vi "Indexer.vi"() -> ()   [LabVIEW 2020]
doc: "Use this template to build a producer/consumer design pattern with events to produce queue items. Use this design pattern instead of the User Interface Event Handler pattern for user interfaces when you want to execute code asynchronously in response to an event without slowing the user interface responsiveness."
uses:
  Model/AbstractModel/AbstractModel.lvclass
  Model/MarkovModel/MarkovModel.lvclass
  C:/Projects/DMC/DMC-Complete/Model/AbstractModel/AbstractModel.lvclass
  DBMap/DBMap.lvclass
  DBSet/DBSet.lvclass
  Indexer Action.ctl
  File Metadata.ctl
  Node.ctl
  Source to Sink Array.ctl
  File Data.ctl
panel:
  out "data":T5
  in  "Tab Control":enum32{"Main", "Debug"}(tab)
  in  "Download Pre-Index Button":bool
  out "# of files":i32 format="%d files"
  out "Markov Progress":u64(slide) scale=-1.0..4743.0
  out "Saving model to file":bool
  in  "Run Training":bool
  in  "Training Folders":path[](array[path])
  in  "Load Example Paths":bool
  out "Pulling training files":bool
  out "Converting to node-child maps":bool
  out "Training model":bool
  out "Node Progress":u64(slide) scale=-1.0..10515.0
  in  "stop":bool
  in  "Load from file":bool
  in  "Save to file":bool
  in  "Stage 3 - Train Model":bool
  in  "Stage 1 - Pull Example Files":bool
  in  "Stage 2 - Convert to Node-Child Maps":bool
  in  "Parallel Instances":i32=8
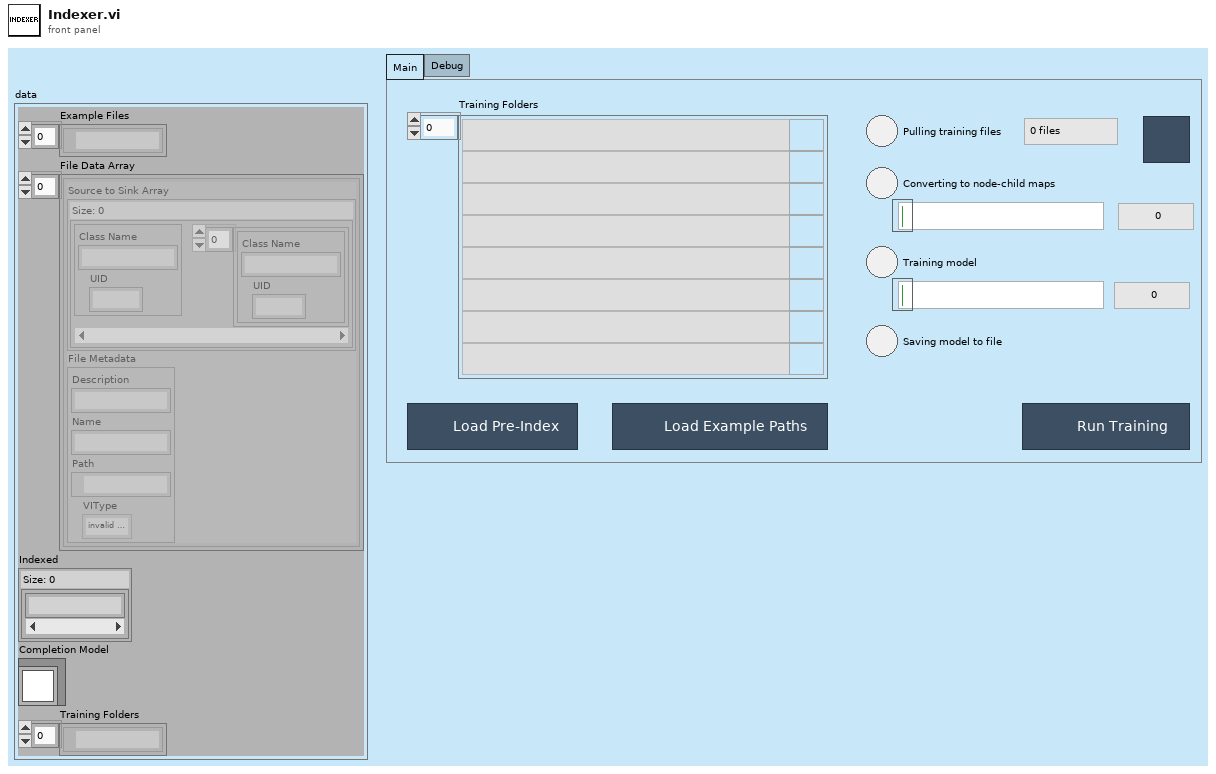
[diagram p1: front panel]
types:
  T1 = typedef "File Data.ctl" = cluster{"Source to Sink Array":T2, "File Metadata":T4}
  T2 = typedef "Source to Sink Array.ctl" = map{T3, T3[]}
  T3 = typedef "Node.ctl" = cluster{"Class Name":string, "UID":i32}
  T4 = typedef "File Metadata.ctl" = cluster{"Description":string, "Name":string, "Path":path, "VIType":enum32{"invalid VI type", "Standard VI", "Control VI", "Global VI", "Polymorphic VI", "Configuration VI", "SubSystem", "Facade VI", "Method VI", "Statechart Diagram VI"}}
  T5 = cluster{"Example Files":path[], "File Data Array":T1[], "Indexed":set{string}, "Completion Model":refnum<class "AbstractModel.lvclass">, "Training Folders":path[]}
  T6 = typedef "Indexer Action.ctl" = enum16{"Pull Training Files", "Convert to Node-Child Maps", "Train Model", "Save to file", "Load from file", "Load Example Paths", "Download Pre-Index"}
  T7 = enum8{"Enabled", "Disabled", "Disabled and Grayed Out"}
  T8 = cluster{"Example Files":path[], "File Data Array":T1[], "Indexed":set{string}, "MarkovModel out":refnum<class "MarkovModel.lvclass">, "Training Folders":path[]}
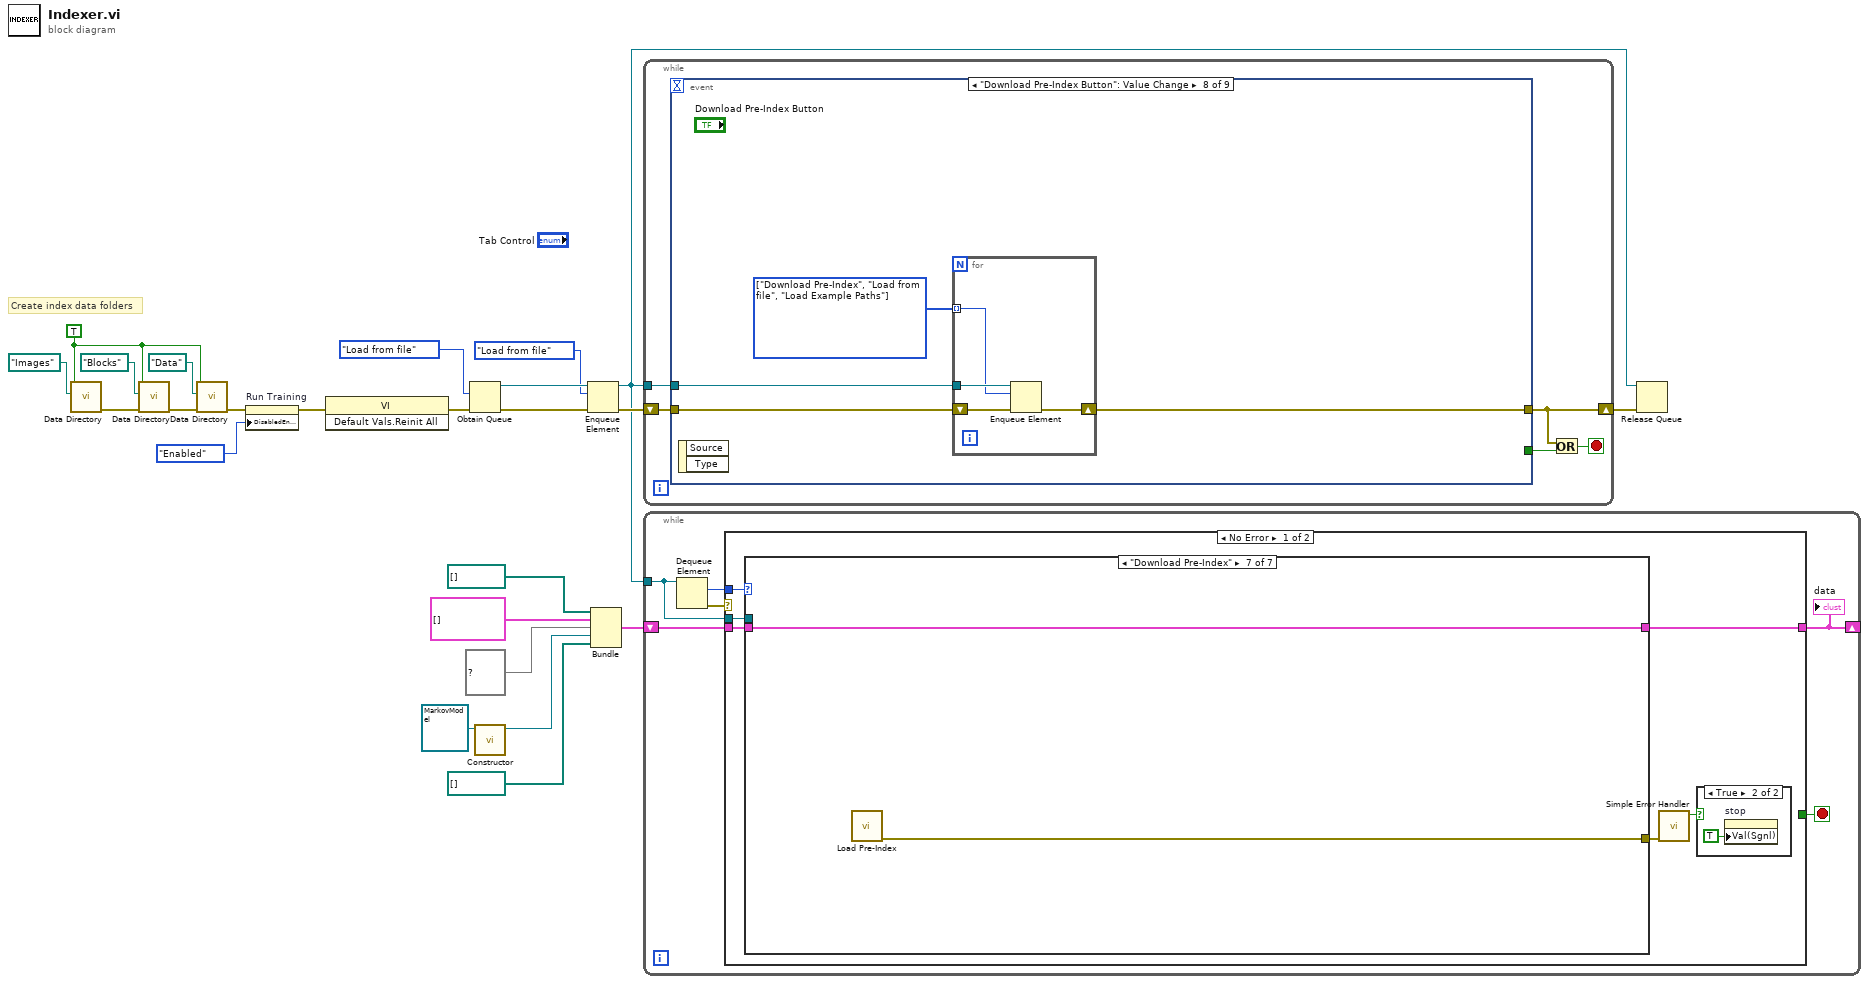
[diagram p0: block diagram]
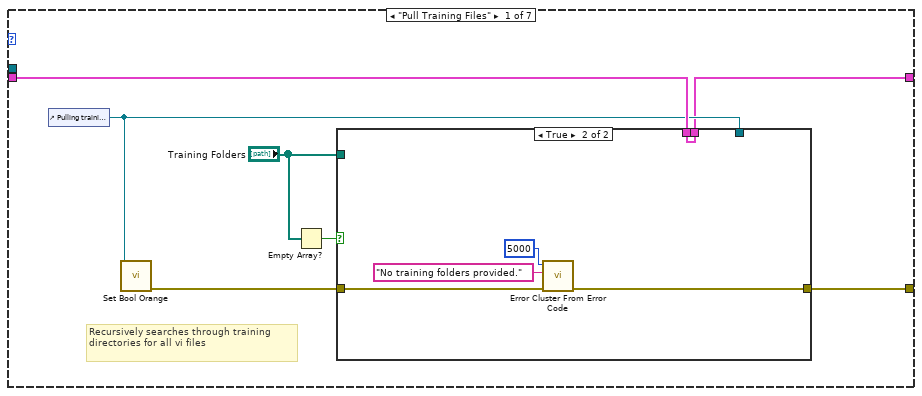
[diagram p2: hidden frame]
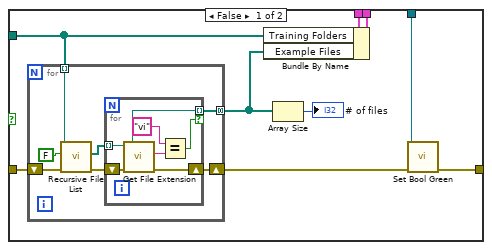
[diagram p3: hidden frame]
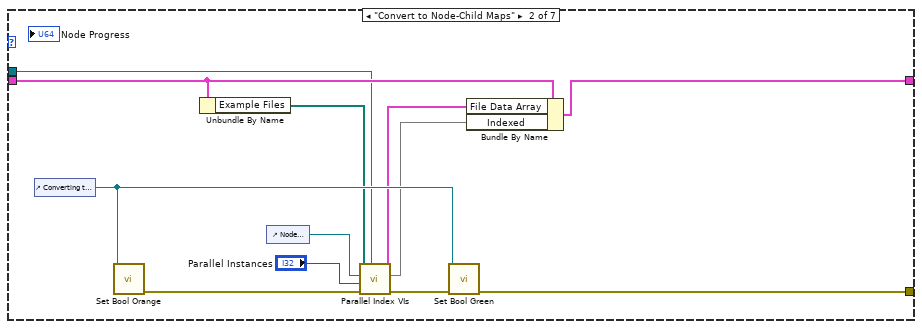
[diagram p4: hidden frame]
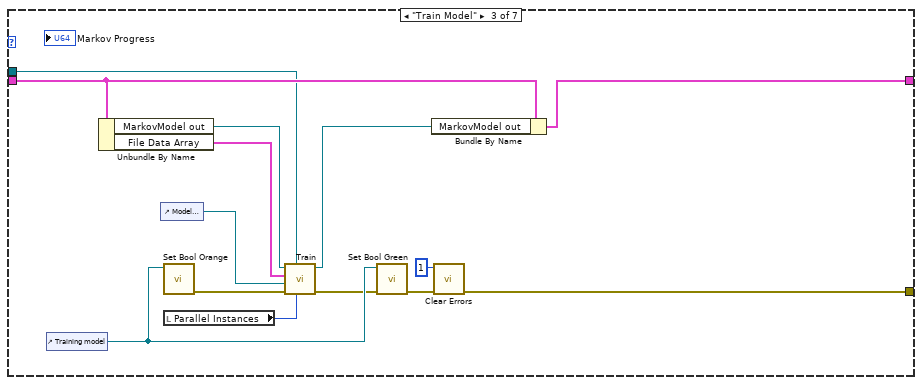
[diagram p5: hidden frame]
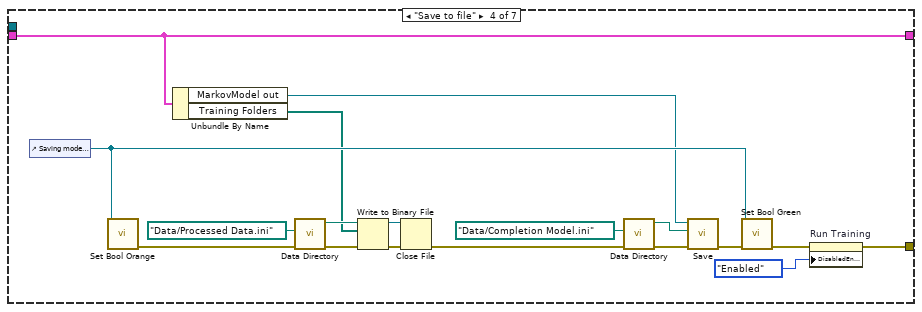
[diagram p6: hidden frame]
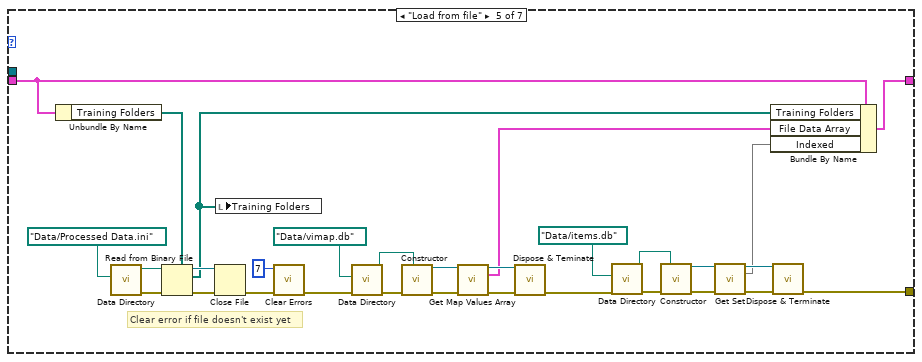
[diagram p7: hidden frame]
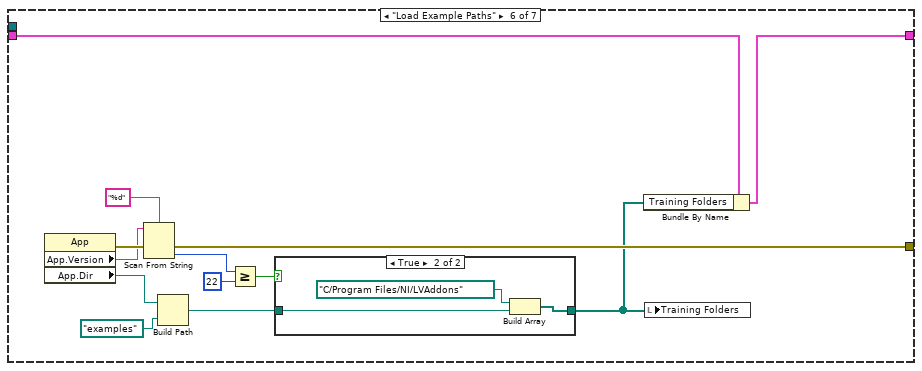
[diagram p8: hidden frame]
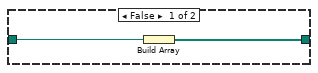
[diagram p9: hidden frame]
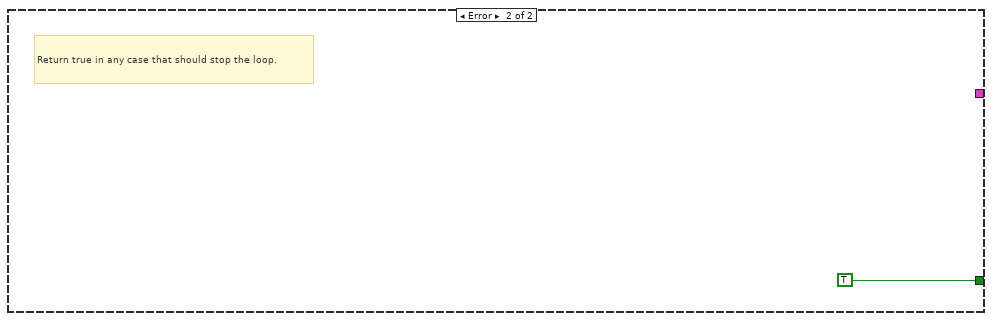
[diagram p11: hidden frame]
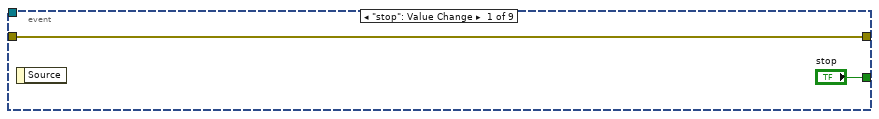
[diagram p12: hidden frame]
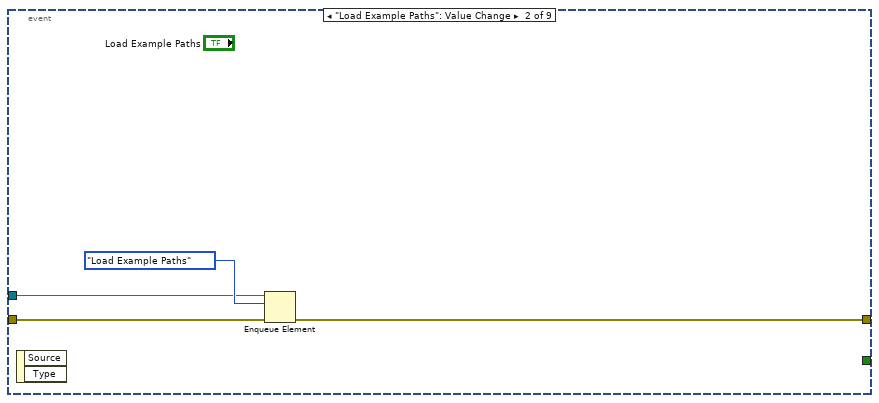
[diagram p13: hidden frame]
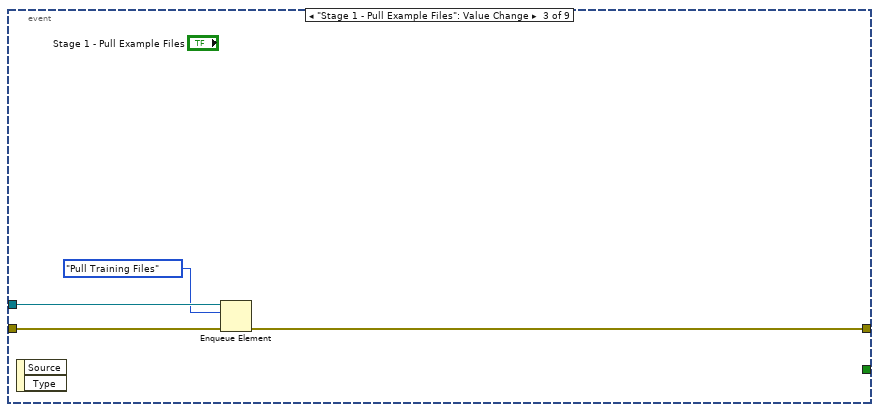
[diagram p14: hidden frame]
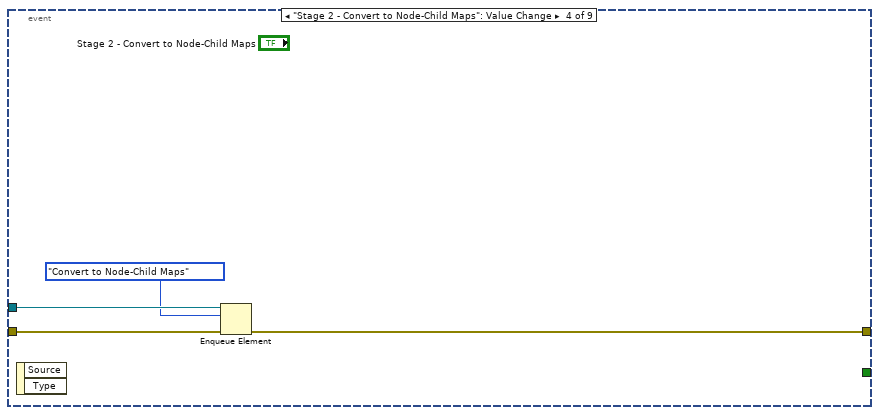
[diagram p15: hidden frame]
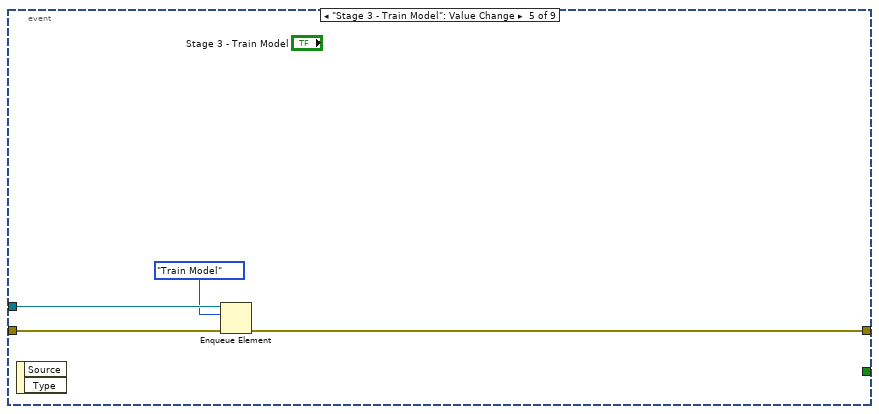
[diagram p16: hidden frame]
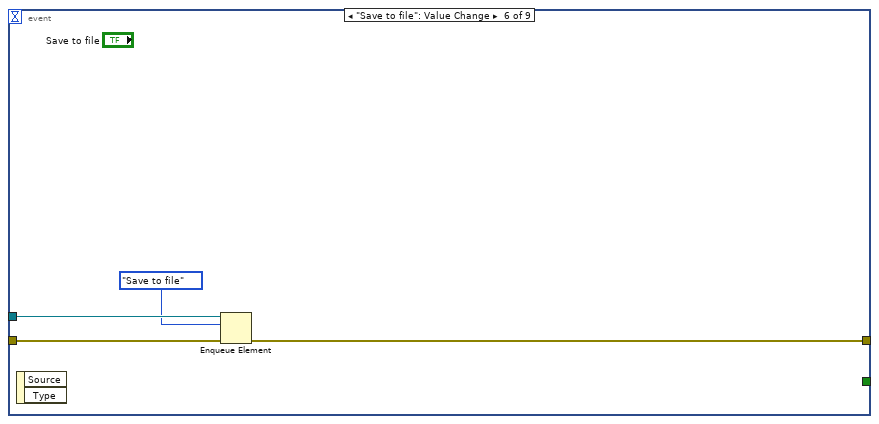
[diagram p17: hidden frame]
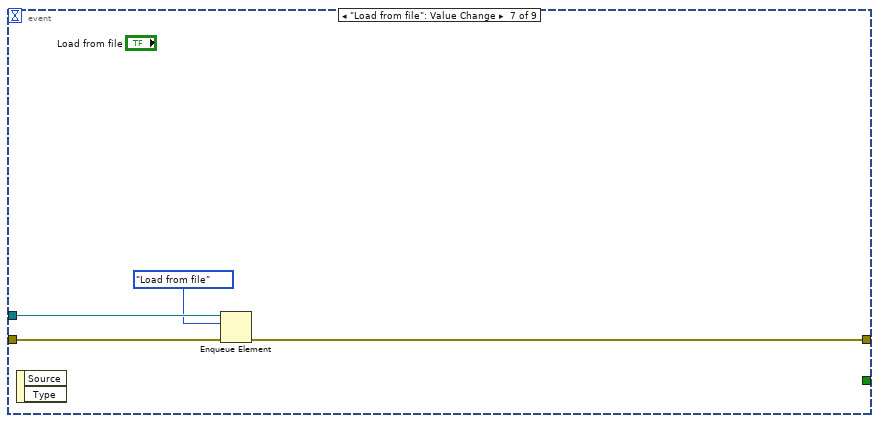
[diagram p18: hidden frame]
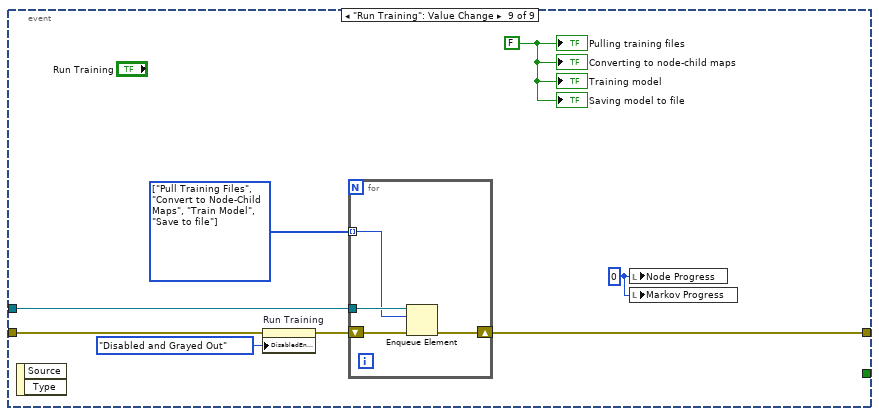
[diagram p19: hidden frame]
diagram:
  w5 = TRUE ("Create if doesn't exist? (F)")
  # "Create index data folders"
  n1 = call "Data Directory.vi"("Subdirectory"=path "Images" ("name or relative path"), "Create if doesn't exist? (F)"=w5) -> ("error out"=w6:errorcluster)  [unwired: 8 in, 1 out]
  n2 = call "Data Directory.vi"("error in (no error)"=w6, "Subdirectory"=path "Blocks" ("name or relative path"), "Create if doesn't exist? (F)"=w5) -> ("error out"=w7:errorcluster)  [unwired: 7 in, 1 out]
  n3 = call "Data Directory.vi"("error in (no error)"=w7, "Subdirectory"=path "Data" ("name or relative path"), "Create if doesn't exist? (F)"=w5) -> ("error out"=w4:errorcluster)  [unwired: 7 in, 1 out]
  n4 = property on="Run Training" class="Bool"(error in=w4, "DisabledEnum"=T7."Enabled") -> (error out=w12:errorcluster)  [unwired: 1 in, 1 out]
  n5 = invoke class="VI" method="Default Vals.Reinit All"(error in=w12) -> (error out=w14:errorcluster)  [unwired: 2 in, 2 out]
  n6 = Obtain Queue(element data type=Indexer_Action."Load from file" ("Indexer Action"), error in (no error)=w14) -> (queue out=w17:refnum<queue>, error out=w19:errorcluster)  [unwired: 3 in, 1 out]
  n7 = call-dynamic "Constructor.vi"("MarkovModel in"=refnum<class "MarkovModel.lvclass"> refnum ("MarkovModel.lvclass")) -> ("MarkovModel out"=w1:refnum<class "MarkovModel.lvclass">)  [unwired: 9 in, 1 out]
  n8 = Enqueue Element(queue=w17, element=Indexer_Action."Load from file", error in (no error)=w19) -> (queue out=w15:refnum<queue>, error out=w18:errorcluster)  [unwired: 1 in, 1 out]
  n9 = Bundle("Example Files"=path[] [], "File Data Array"=T1[] [], "Indexed"=set{string} {}, "MarkovModel out"=w1, "Training Folders"=path[] []) -> (w20:T8)  [unwired: 1 in]
  n10 = while {
    shift-right: [w25] -> w24
    shift-left: w18 -> [w28]
    tunnel: w15 -> [w29]
    stop <- w26 stop-if-true
    n11 = event shown="[7] \"Download Pre-Index Button\": Value Change" {
      selector: _ -> [_ _ _ _ _ _ _ _ _]
      dyn-events: _ -> [_ _ _ _ _ _ _ _ _]
      timeout: _ -> [_ _ _ _ _ _ _ _ _]
      tunnel: w29 -> [_ w32 w38 w42 w46 w50 w54 w57 w71]
      tunnel: w28 -> [w30 w34 w39 w43 w47 w51 w55 w59 w67]
      tunnel: [w30 w33 w37 w41 w45 w49 w53 w58 w70] -> w25
      tunnel: ["stop" _ _ _ _ _ _ _ _] -> w27
      event "stop": Value Change {
        n12 = event-data() -> ()  [unwired: 1 in, 1 out]
      }
      event "Load Example Paths": Value Change {
        n13 = event-data() -> ()  [unwired: 1 in, 2 out]
        n14 = Enqueue Element(queue=w32, element=Indexer_Action."Load Example Paths" ("Indexer Action"), error in (no error)=w34) -> (error out=w33:errorcluster)  [unwired: 1 in, 2 out]
      }
      event "Stage 1 - Pull Example Files": Value Change {
        n15 = event-data() -> ()  [unwired: 1 in, 2 out]
        n16 = Enqueue Element(queue=w38, element=Indexer_Action."Pull Training Files" ("Indexer Action"), error in (no error)=w39) -> (error out=w37:errorcluster)  [unwired: 1 in, 2 out]
      }
      event "Stage 2 - Convert to Node-Child Maps": Value Change {
        n17 = event-data() -> ()  [unwired: 1 in, 2 out]
        n18 = Enqueue Element(queue=w42, element=Indexer_Action."Convert to Node-Child Maps" ("Indexer Action"), error in (no error)=w43) -> (error out=w41:errorcluster)  [unwired: 1 in, 2 out]
      }
      event "Stage 3 - Train Model": Value Change {
        n19 = event-data() -> ()  [unwired: 1 in, 2 out]
        n20 = Enqueue Element(queue=w46, element=Indexer_Action."Train Model" ("Indexer Action"), error in (no error)=w47) -> (error out=w45:errorcluster)  [unwired: 1 in, 2 out]
      }
      event "Save to file": Value Change {
        n21 = event-data() -> ()  [unwired: 1 in, 2 out]
        n22 = Enqueue Element(queue=w50, element=Indexer_Action."Save to file" ("Indexer Action"), error in (no error)=w51) -> (error out=w49:errorcluster)  [unwired: 1 in, 2 out]
      }
      event "Load from file": Value Change {
        n23 = event-data() -> ()  [unwired: 1 in, 2 out]
        n24 = Enqueue Element(queue=w54, element=Indexer_Action."Load from file" ("Indexer Action"), error in (no error)=w55) -> (error out=w53:errorcluster)  [unwired: 1 in, 2 out]
      }
      event "Download Pre-Index Button": Value Change {
        w56 = T6[] [enum."Download Pre-Index", enum."Load from file", enum."Load Example Paths"] items=["Pull Training Files", "Convert to Node-Child Maps", "Train Model", "Save to file", "Load from file", "Load Example Paths", "Download Pre-Index"] ("Array")
        n25 = event-data() -> ()  [unwired: 1 in, 2 out]
        n26 = for {
          tunnel: w57 -> [w62]
          tunnel: w56 -> [w60] mode=indexing
          shift-right: [w61] -> w58
          shift-left: w59 -> [w63]
          n27 = Enqueue Element(queue=w62, element=w60, error in (no error)=w63) -> (error out=w61:errorcluster)  [unwired: 1 in, 2 out]
        }
      }
      event "Run Training": Value Change {
        w64 = u64 0 ("Node Progress")
        w65 = FALSE ("Pulling training files")
        w69 = T6[] [enum."Pull Training Files", enum."Convert to Node-Child Maps", enum."Train Model", enum."Save to file"] items=["Pull Training Files", "Convert to Node-Child Maps", "Train Model", "Save to file", "Load from file", "Load Example Paths", "Download Pre-Index"] ("Array")
        n28 = event-data() -> ()  [unwired: 1 in, 2 out]
        n29 = property on="Run Training" class="Bool"(error in=w67, "DisabledEnum"=T7."Disabled and Grayed Out" ("Disabled")) -> (error out=w68:errorcluster)  [unwired: 1 in, 1 out]
        n30 = for {
          tunnel: w71 -> [w74]
          tunnel: w69 -> [w72] mode=indexing
          shift-right: [w73] -> w70
          shift-left: w68 -> [w75]
          n31 = Enqueue Element(queue=w74, element=w72, error in (no error)=w75) -> (error out=w73:errorcluster)  [unwired: 1 in, 2 out]
        }
        n32 = local write "Node Progress"(w64) -> ()
        n33 = local write "Markov Progress"(w64) -> ()
        "Converting to node-child maps" <- w65
        "Training model" <- w65
        "Pulling training files" <- w65
        "Saving model to file" <- w65
      }
    }
    n34 = Or(x=w25, y=w27) -> (x .or. y?=w26:bool)
  }
  n35 = while {
    tunnel: w15 -> [w77]
    shift-right: [w76] -> _
    shift-left: w20 -> [w78]
    stop <- w79 stop-if-true
    n36 = Dequeue Element(queue=w77) -> (element=w80:T6, error out=w81:errorcluster)  [unwired: 2 in, 2 out]
    n37 = case shown="No Error" w81 {
      tunnel: w80 -> [w87 _]
      tunnel: [_ TRUE] -> w79
      tunnel: w78 -> [w86 _]
      tunnel: [w85 _] -> w76
      tunnel: w77 -> [w84 _]
      frame No Error {
        n38 = case shown="\"Download Pre-Index\"" w87 {
          tunnel: [w88 w122 w134 w151 w186 w197 w214] -> w85
          tunnel: w86 -> [w94 w133 w146 w151 w188 w198 w214]
          tunnel: w84 -> [_ w127 w140 _ _ _ _]
          tunnel: [w92 w131 w144 w160 w166 w200 w215] -> w83
          frame "Pull Training Files" {
            # "Recursively searches through training directories for all vi files"
            n39 = control-ref of="Pulling training files"() -> (w91:refnum<vi>)
            n40 = call "Set Bool Orange.vi"("Indicator ref in"=w91) -> ("error out"=w93:errorcluster)  [unwired: 10 in]
            n41 = Empty Array?(array="Training Folders") -> (empty?=w89:bool)
            n42 = case shown="True" w89 {
              tunnel: w94 -> [w103 w121]
              tunnel: [w102 w121] -> w88
              tunnel: w93 -> [w101 w120]
              tunnel: [w99 w119] -> w92
              tunnel: w91 -> [w98 _]
              tunnel: "Training Folders" -> [w95 _]
              frame False {
                n43 = for {
                  tunnel: w95 -> [w110] mode=indexing
                  shift-right: [w105] -> w100
                  shift-left: w101 -> [w106]
                  tunnel: [w104] -> w97 mode=concatenating
                  n44 = call <vilib>:"Recursive File List.vi"("error in (no error)"=w106, "Treat LLBs as Folders?"=FALSE, "Folder Path"=w110) -> ("error out"=w107:errorcluster, "All Files in Dir"=w108:path[])  [unwired: 4 in, 3 out]
                  n45 = for {
                    tunnel: w108 -> [w113] mode=indexing
                    tunnel: [w113] -> w104 mode=indexing if=w112
                    shift-right: [w111] -> w105
                    shift-left: w107 -> [w116]
                    n46 = call <vilib>:"Get File Extension.vi"("error in (no error)"=w116, "file"=w113) -> ("error out"=w111:errorcluster, "lowercase file extension"=w114:string)  [unwired: 5 in, 3 out]
                    n47 = Equal?(x="vi", y=w114) -> (x = y?=w112:bool)
                  }
                }
                n48 = Bundle By Name(cluster=w103, "Training Folders"=w95, "Example Files"=w97) -> (w102:T8)
                n49 = Array Size(array=w97) -> (size(s)=→"# of files":i32)
                n50 = call "Set Bool Green.vi"("error in (no error)"=w100, "Indicator ref in"=w98) -> ("error out"=w99:errorcluster)  [unwired: 9 in]
              }
              frame True {
                n51 = call <vilib>:"Error Cluster From Error Code.vi"("error in (no error)"=w120, "error message (\"\")"="No training folders provided." ("error message (\"\")"), "error code (0)"=5000) -> ("error out"=w119:errorcluster)  [unwired: 6 in]
              }
            }
          }
          frame "Convert to Node-Child Maps" {
            n52 = control-ref of="Converting to node-child maps"() -> (w130:refnum<vi>)
            n53 = call "Set Bool Orange.vi"("Indicator ref in"=w130) -> ("error out"=w132:errorcluster)  [unwired: 10 in]
            n54 = Unbundle By Name(w133) -> ("Example Files"=w128:path[])
            n55 = control-ref of="Node Progress"() -> (w126:refnum<vi>)
            n56 = call "Parallel Index VIs.vi"("Queue in"=w127, "error in (no error)"=w132, "Parallel Instances (8)"="Parallel Instances", "Node Progress ref"=w126, "Example Files"=w128) -> ("error out"=w129:errorcluster, "Indexed"=w125:set{string}, "File Data Array"=w123:T1[])  [unwired: 4 in]
            n57 = call "Set Bool Green.vi"("error in (no error)"=w129, "Indicator ref in"=w130) -> ("error out"=w131:errorcluster)  [unwired: 9 in]
            n58 = Bundle By Name(cluster=w133, "File Data Array"=w123, "Indexed"=w125) -> (w122:T8)
          }
          frame "Train Model" {
            n59 = control-ref of="Training model"() -> (w147:refnum<vi>)
            n60 = Unbundle By Name(w146) -> ("MarkovModel out"=w139:refnum<class "MarkovModel.lvclass">, "File Data Array"=w138:T1[])
            n61 = control-ref of="Model Progress"() -> (w137:refnum<vi>)
            n62 = call "Set Bool Orange.vi"("Indicator ref in"=w147) -> ("error out"=w142:errorcluster)  [unwired: 10 in]
            n63 = local read "Parallel Instances"() -> (w136:i32)
            n64 = call-dynamic "Train.vi"("Parallel Instances (8)"=w136, "Queue in"=w140, "error in (no error)"=w142, "Progress ref in"=w137, "File Data Array"=w138, "MarkovModel in"=w139) -> ("error out"=w141:errorcluster, "MarkovModel out"=w135:refnum<class "MarkovModel.lvclass">)  [unwired: 4 in]
            n65 = call "Set Bool Green.vi"("error in (no error)"=w141, "Indicator ref in"=w147) -> ("error out"=w145:errorcluster)  [unwired: 9 in]
            n66 = Bundle By Name(cluster=w146, "MarkovModel out"=w135) -> (w134:T8)
            n67 = call <vilib>:"Clear Errors.vi"("error in (no error)"=w145, "specific error code to clear (0: all)"=1) -> ("error out"=w144:errorcluster)  [unwired: 4 in, 1 out]
          }
          frame "Save to file" {
            n68 = control-ref of="Saving model to file"() -> (w163:refnum<vi>)
            n69 = call "Set Bool Orange.vi"("Indicator ref in"=w163) -> ("error out"=w149:errorcluster)  [unwired: 10 in]
            n70 = Unbundle By Name(w151) -> ("MarkovModel out"=w156:refnum<class "MarkovModel.lvclass">, "Training Folders"=w150:path[])
            n71 = call "Data Directory.vi"("error in (no error)"=w149, "Subdirectory"=path "Data/Processed Data.ini" ("name or relative path")) -> ("error out"=w148:errorcluster, "Data directory"=w158:path)  [unwired: 8 in]
            n72 = Write to Binary File(file (use dialog)=w158, data=w150, error in=w148) -> (refnum out=w164:refnum<file>, error out=w165:errorcluster)  [unwired: 3 in, 1 out]
            n73 = Close File(refnum=w164, error in=w165) -> (error out=w153:errorcluster)  [unwired: 1 out]
            n74 = call "Data Directory.vi"("error in (no error)"=w153, "Subdirectory"=path "Data/Completion Model.ini" ("name or relative path")) -> ("error out"=w152:errorcluster, "Data directory"=w154:path)  [unwired: 8 in]
            n75 = call-dynamic "Save.vi"("error in (no error)"=w152, "Model Path"=w154, "MarkovModel in"=w156) -> ("error out"=w157:errorcluster)  [unwired: 7 in, 1 out]
            n76 = call "Set Bool Green.vi"("error in (no error)"=w157, "Indicator ref in"=w163) -> ("error out"=w161:errorcluster)  [unwired: 9 in]
            n77 = property on="Run Training" class="Bool"(error in=w161, "DisabledEnum"=T7."Enabled" ("Disabled")) -> (error out=w160:errorcluster)  [unwired: 1 in, 1 out]
          }
          frame "Load from file" {
            # "Clear error if file doesn't exist yet"
            n78 = Unbundle By Name(w188) -> ("Training Folders"=w187:path[])
            n79 = call "Data Directory.vi"("Subdirectory"=path "Data/Processed Data.ini" ("name or relative path")) -> ("error out"=w189:errorcluster, "Data directory"=w190:path)  [unwired: 9 in]
            n80 = Read from Binary File(5:w187, 8:w189, 11:w190) -> (0:w195:errorcluster, 2:w185:path[], 3:w194:refnum<file>)  [unwired: 3 in, 1 out]
            n81 = Close File(refnum=w194, error in=w195) -> (error out=w193:errorcluster)  [unwired: 1 out]
            n82 = local write "Training Folders"(w185) -> ()
            n83 = call <vilib>:"Clear Errors.vi"("error in (no error)"=w193, "specific error code to clear (0: all)"=7) -> ("error out"=w178:errorcluster)  [unwired: 4 in, 1 out]
            n84 = call "Data Directory.vi"("error in (no error)"=w178, "Subdirectory"=path "Data/vimap.db" ("name or relative path")) -> ("error out"=w183:errorcluster, "Data directory"=w182:path)  [unwired: 8 in]
            n85 = call "Constructor.vi"("SQLite DB Path"=w182, "error in (no error)"=w183) -> ("error out"=w176:errorcluster, "DBMap out"=w177:refnum<class "DBMap.lvclass">)  [unwired: 8 in]
            n86 = call "Get Map Values Array.vi"("DBMap in"=w177, "error in (no error)"=w176) -> ("DBMap out"=w174:refnum<class "DBMap.lvclass">, "File Data Array"=w172:T1[], "error out"=w175:errorcluster)  [unwired: 11 in]
            n87 = call-dynamic "Dispose & Teminate.vi"("DBMap in"=w174, "error in (no error)"=w175) -> ("error out"=w173:errorcluster)  [unwired: 12 in, 1 out]
            n88 = call "Data Directory.vi"("error in (no error)"=w173, "Subdirectory"=path "Data/items.db" ("name or relative path")) -> ("error out"=w180:errorcluster, "Data directory"=w179:path)  [unwired: 8 in]
            n89 = call "Constructor.vi"("SQLite DB Path"=w179, "error in (no error)"=w180) -> ("DBSet out"=w168:refnum<class "DBSet.lvclass">, "error out"=w171:errorcluster)  [unwired: 12 in]
            n90 = call "Get Set.vi"("DBSet in"=w168, "error in (no error)"=w171) -> ("DBSet out"=w169:refnum<class "DBSet.lvclass">, "Set"=w167:set{string}, "error out"=w170:errorcluster)  [unwired: 11 in]
            n91 = Bundle By Name(cluster=w188, "Training Folders"=w185, "File Data Array"=w172, "Indexed"=w167) -> (w186:T8)
            n92 = call-dynamic "Dispose & Terminate.vi"("DBSet in"=w169, "error in (no error)"=w170) -> ("error out"=w166:errorcluster)  [unwired: 12 in, 1 out]
          }
          frame "Load Example Paths" {
            n93 = property class="App"() -> (error out=w203:errorcluster, "App.Version"=w199:string, "App.Dir"=w204:path)  [unwired: 2 in, 1 out]
            n94 = Scan From String(format string="%d", input string=w199, error in=w203) -> (error out=w200:errorcluster, output 1=w206:i32)  [unwired: 2 in, 2 out]
            n95 = Build Path(base path=w204, name or relative path=path "examples" ("Path")) -> (appended path=w201:path)
            n96 = Greater Or Equal?(x=w206, y=22) -> (x >= y?=w202:bool)
            n97 = case shown="True" w202 {
              tunnel: w201 -> [w210 w213]
              tunnel: [w209 w212] -> w196
              frame False {
                n98 = Build Array(w210) -> (w209:path[])
              }
              frame True {
                n99 = Build Array(path "C:/Program Files/NI/LVAddons" ("Path"), w213) -> (w212:path[])
              }
            }
            n100 = Bundle By Name(cluster=w198, "Training Folders"=w196) -> (w197:T8)
            n101 = local write "Training Folders"(w196) -> ()
          }
          frame "Download Pre-Index" {
            n102 = call "Load Pre-Index.vi"() -> ("error out"=w215:errorcluster)  [unwired: 11 in]
          }
        }
        n103 = call <vilib>:"Simple Error Handler.vi"("error in (no error)"=w83) -> ("error?"=w82:bool)  [unwired: 4 in, 4 out]
        n104 = case shown="True" w82 {
          frame False {
          }
          frame True {
            n105 = property on="stop" class="Bool (strict)"("Val(Sgnl)"=TRUE ("Value (Signaling)")) -> ()  [unwired: 2 in, 2 out]
          }
        }
      }
      frame Error {
        # "Return true in any case that should stop the loop."
      }
    }
    "data" <- w76
  }
  n106 = Release Queue(queue=w15, error in (no error)=w24) -> ()  [unwired: 1 in, 3 out]
